vi "_ValidateDeviceProfiles.vi"(8 "error in (no error)":errorcluster, 9 "ddSrcPath":string[](array[string]), 10 "reference in":refnum<vi>) -> (0 "error out":errorcluster, 1 "profileImport":T1[](array[typedef]), 2 "reference out":refnum<vi>)   [LabVIEW 2020, in "SEECD System Explorer.lvlib"]
uses:
  SEECD System Explorer.lvlib
  <resource>/Framework/Providers/indcomecat/_InternalSubVIs/_profileImport.ctl
  Applications/Utilities/ECAT Files.ctl
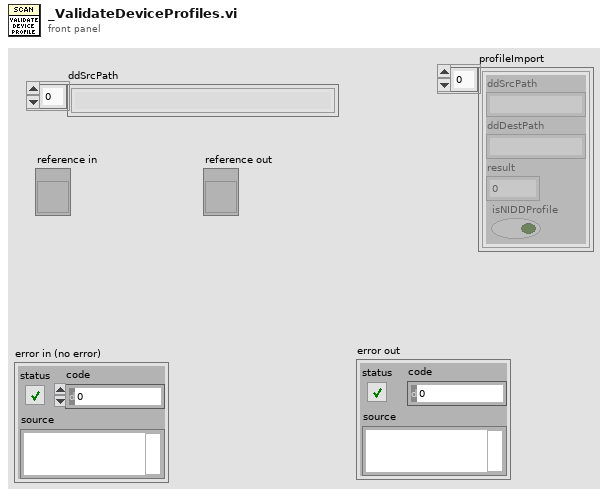
[diagram p1: front panel]
types:
  T1 = typedef "_profileImport.ctl" = cluster{"ddSrcPath":string, "ddDestPath":string, "result":i32, "isNIDDProfile":bool}
  T2 = typedef "SEECD System Explorer.lvlib/ECAT Files.ctl" = enum16{"niECATLVProvider.mxx", "indcomecat.chm", "Providers DD", "Shared DD"}
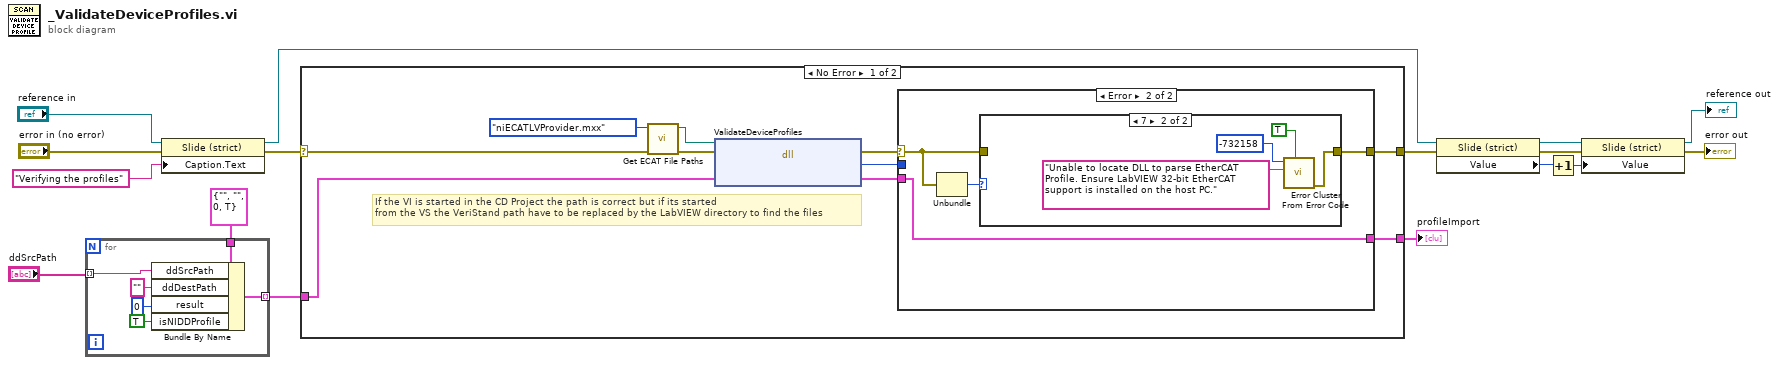
[diagram p0: block diagram]
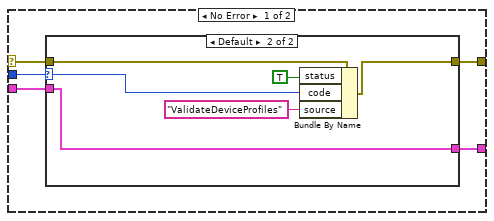
[diagram p2: hidden frame]
diagram:
  n1 = for {
    tunnel: "ddSrcPath" -> [w21] mode=indexing
    tunnel: [w22] -> w14 mode=indexing
    tunnel: T1 {"ddSrcPath"="", "ddDestPath"="", "result"=0, "isNIDDProfile"=TRUE} ("input cluster") -> [w20]
    n2 = Bundle By Name(cluster=w20, "ddSrcPath"=w21, "ddDestPath"="" ("ddRootPath"), "result"=0, "isNIDDProfile"=TRUE) -> (w22:T1)
  }
  n3 = property class="Slide (strict)"(reference="reference in", error in="error in (no error)", "Caption.Text"="Verifying the profiles") -> (reference out=w1:refnum<vi>, error out=w11:errorcluster)
  n4 = case shown="No Error" w11 {
    selector: w11 -> [w26 w56]
    tunnel: [w30 w56] -> w8
    tunnel: w14 -> [w27 w55]
    tunnel: [w28 w55] -> w13
    frame No Error {
      # "If the VI is started in the CD Project the path is correct but if its started \nfrom the VS the VeriStand path have to be replaced by the LabVIEW directory to find the files"
      n5 = call "Get ECAT File Paths.vi"("error in"=w26, "ECAT File"=ECAT_Files."niECATLVProvider.mxx") -> ("error out"=w25:errorcluster, "File Path"=w24:path)  [unwired: 8 in]
      n6 = dll-call lib="C:/Users/grschero/Desktop/CD-Project Folder/CD_Project/Scan-Engine-Custom-Device_EtherCAT_AKD_Extension/Scan-Engine-Custom-Device/Custom Device Source/niECATLVProvider.mxx" fn="ValidateDeviceProfiles"(path in=w24, error in=w25, "profileImport"=w27) -> (error out=w29:errorcluster, "return type"=w31:i32, "profileImport"=w32:T1[])  [unwired: 1 in, 1 out]
      n7 = case shown="Error" w29 {
        selector: w29 -> [w34 w47]
        tunnel: w32 -> [w37 w49]
        tunnel: w31 -> [w36 _]
        tunnel: [w35 w46] -> w30
        tunnel: [w33 w49] -> w28
        frame No Error {
          n8 = case shown="Default" w36 {
            selector: w36 -> [_ w45]
            tunnel: [w39 w42] -> w35
            tunnel: w34 -> [w39 w41]
            tunnel: w37 -> [w38 w40]
            tunnel: [w38 w40] -> w33
            frame 0 {
            }
            frame Default {
              n9 = Bundle By Name(cluster=w41, "status"=TRUE, "code"=w45, "source"="ValidateDeviceProfiles") -> (w42:errorcluster)
            }
          }
        }
        frame Error {
          n10 = Unbundle(w47) -> ("code"=w48:i32)  [unwired: 2 out]
          n11 = case shown="7" w48 {
            tunnel: w47 -> [w50 _]
            tunnel: [w50 w54] -> w46
            frame Default {
            }
            frame 7 {
              n12 = call <vilib>:"Error Cluster From Error Code.vi"("show call chain? (False)"=TRUE, "error message (\"\")"="Unable to locate DLL to parse EtherCAT Profile. Ensure LabVIEW 32-bit EtherCAT support is installed on the host PC." ("error message (\"\")"), "error code (0)"=-732158) -> ("error out"=w54:errorcluster)  [unwired: 6 in]
            }
          }
        }
      }
    }
    frame Error {
    }
  }
  "profileImport" <- w13
  n13 = property class="Slide (strict)"(reference=w1, error in=w8) -> (reference out=w4:refnum<vi>, error out=w5:errorcluster, "Value"=w7:u8)
  n14 = Increment(x=w7) -> (x+1=w6:u8)
  n15 = property class="Slide (strict)"(reference=w4, error in=w5, "Value"=w6) -> (reference out=→"reference out":refnum<vi>, error out=→"error out":errorcluster)
